vi "RDC-Lin-Calc_Impedance2.vi"(11 "input cluster":T1) -> (2 "Impedance":cdb[](array[numeric]), 3 "Output cluster":T1)   [LabVIEW 2020, in "RDC-Reflection_Data_Computation.lvlib"]
doc: "Computes the impedance from the reflection of a Common Format cluster and returns it, together with the cluster with Resistance and Reactance filled in."
uses:
  RDC-Reflection_Data_Computation.lvlib
  Reflector/RFH-common_data_format.ctl
  Reflector/RFH-Reflection_File_Handler.lvlib
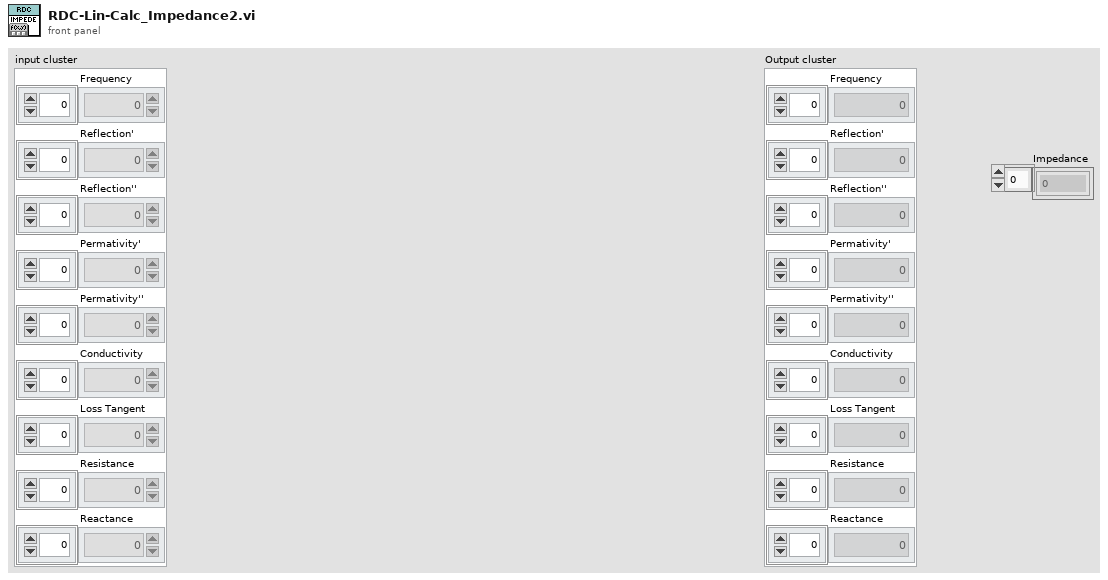
[diagram p1: front panel]
types:
  T1 = typedef "RFH-Reflection_File_Handler.lvlib/RFH-common_data_format.ctl" = cluster{"Frequency":dbl[], "Reflection'":dbl[], "Reflection''":dbl[], "Permativity'":dbl[], "Permativity''":dbl[], "Conductivity":dbl[], "Loss Tangent":dbl[], "Resistance":dbl[], "Reactance":dbl[]}
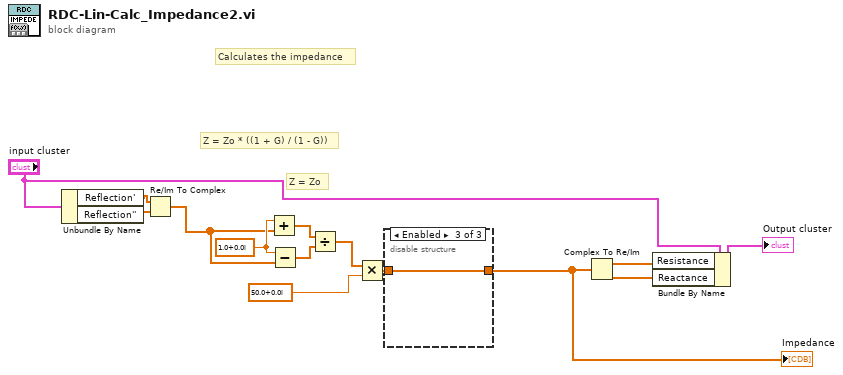
[diagram p0: block diagram]
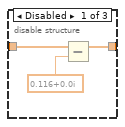
[diagram p2: hidden frame]
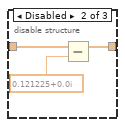
[diagram p3: hidden frame]
diagram:
  w11 = cdb 1.0+0.0i ("x")
  # "Calculates the impedance"
  # "Z = Zo"
  # "Z = Zo * ((1 + G) / (1 - G))"
  n1 = Unbundle By Name("input cluster") -> ("Reflection'"=w8:dbl[], "Reflection''"=w7:dbl[])
  n2 = Re/Im To Complex(1:w7, 2:w8) -> (0:w6:cdb[])
  n3 = Add(x=w11, y=w6) -> (x+y=w12:cdb[])
  n4 = Subtract(x=w11, y=w6) -> (x-y=w13:cdb[])
  n5 = Divide(x=w12, y=w13) -> (x/y=w14:cdb[])
  n6 = Multiply(x=w14, y=cdb 50.0+0.0i) -> (x*y=w9:cdb[])
  n7 = disable-structure shown="Enabled" {
    disable-tunnel: w9 -> [w17 w20 w21]
    disable-tunnel: [w16 w19 w21] -> w4
    frame Disabled {
      n8 = Subtract(x=w17, y=cdb 0.116+0.0i ("x")) -> (x-y=w16:cdb[])
    }
    frame Disabled {
      n9 = Subtract(x=w20, y=cdb 0.121225+0.0i ("x")) -> (x-y=w19:cdb[])
    }
    frame Enabled {
    }
  }
  "Impedance" <- w4
  n10 = Complex To Re/Im(x + iy=w4) -> (x=w2:dbl[], y=w1:dbl[])
  n11 = Bundle By Name(cluster="input cluster", "Resistance"=w2, "Reactance"=w1) -> (→"Output cluster":T1)
